vi "Initialize.vi"(7 "Configure RS232 Baud Rate":u32(ring)=115200 items=["9600"=9600, "19200"=19200, "38400"=38400, "57600"=57600, "115200"=115200], 8 "error in (no error)":errorcluster, 9 "Clear Error(True)":bool=TRUE, 10 "ID Query (True)":bool=TRUE, 11 "VISA resource name":refnum<visa-resource-name>) -> (0 "error out":errorcluster, 1 "ID Return Count":u32, 2 "ID Return String":string, 3 "VISA resource name out":refnum<visa-resource-name>)   [LabVIEW 2012, in "GDM-9052.lvlib"]
doc: "Establishes communication with the instrument and optionally performs an instrument identification query and/or an instrument reset. It also places the instrument in a default state needed for other instrument driver operations. Therefore, call this VI before calling other instrument driver VIs for this instrument. Generally, you need to call the Initialize VI only once at the beginning of an application."
uses:
  GDM-9052.lvlib
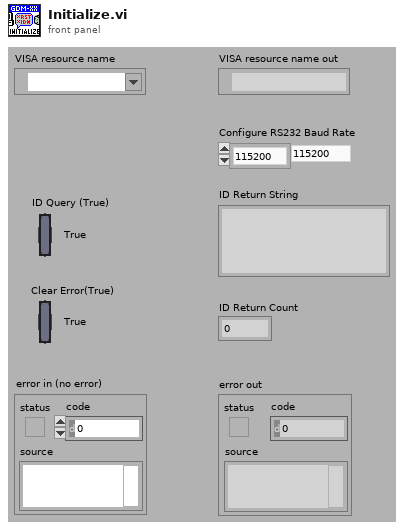
[diagram p1: front panel]
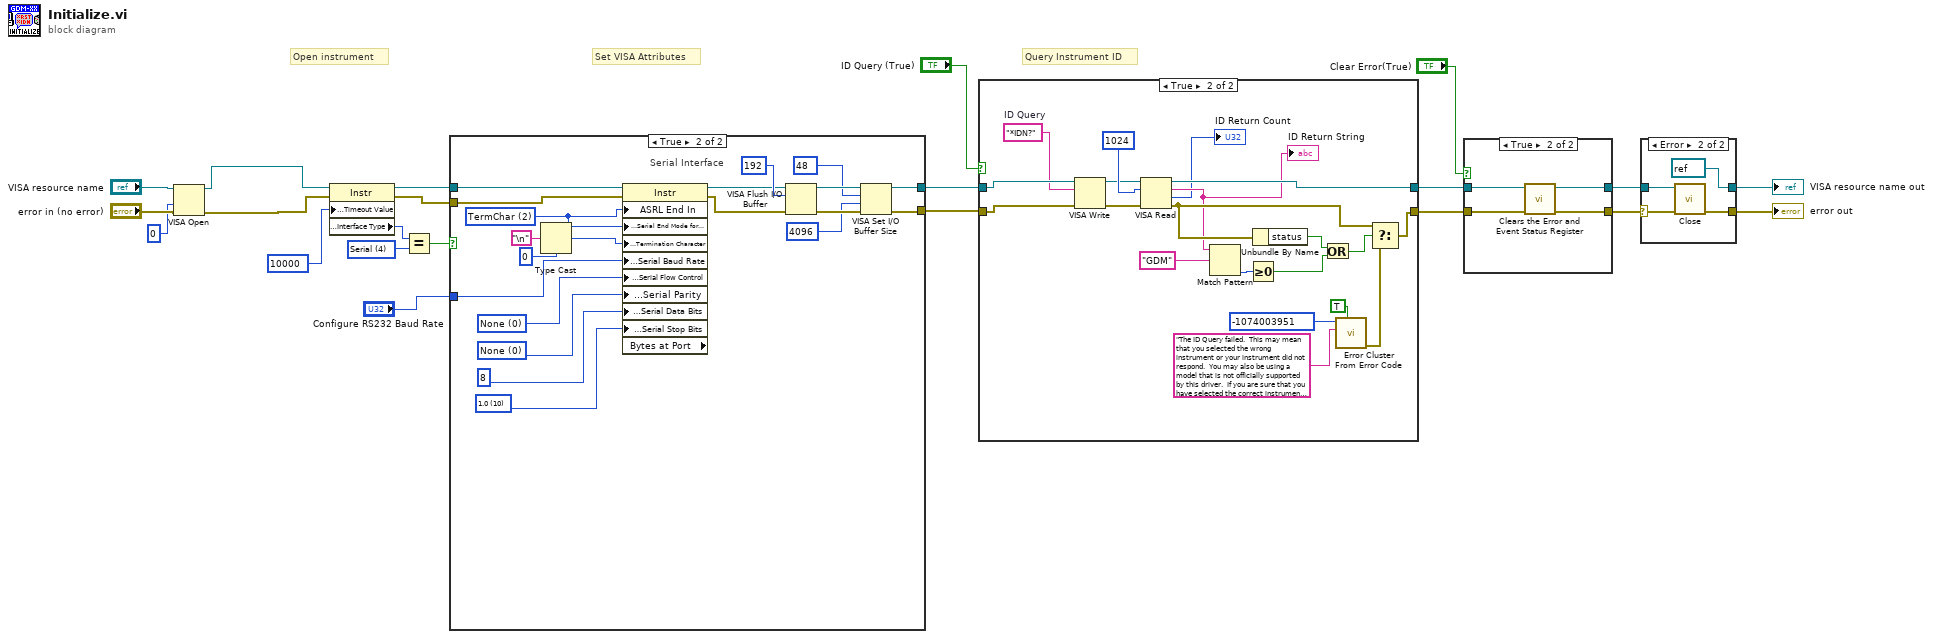
[diagram p0: block diagram]
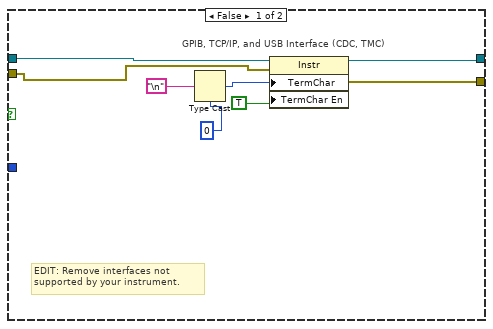
[diagram p4: hidden frame]
diagram:
  w14 = u16 4 items=["GPIB"=1, "VXI"=2, "GPIB-VXI"=3, "Serial"=4, "PXI"=5, "TCPIP"=6, "USB"=7] ("Interface Information:Interface Type")
  # "Set VISA Attributes"
  # "Query Instrument ID"
  # "Open instrument"
  n1 = VISA Open(access mode=u32 0, error in (no error)="error in (no error)", VISA resource name="VISA resource name") -> (VISA resource name=w5:refnum<visa-resource-name>, error out=w4:errorcluster)  [unwired: 2 in]
  n2 = property class="Instr"(reference=w5, error in=w4, "General Settings:Timeout Value"=u32 10000) -> (reference out=w17:refnum<visa-resource-name>, error out=w16:errorcluster, "Interface Information:Interface Type"=w11:u16)
  n3 = Equal?(x=w11, y=w14) -> (x = y?=w15:bool)
  n4 = case shown="True" w15 {
    tunnel: [w26 w32] -> w10
    tunnel: [w25 w31] -> w9
    tunnel: w17 -> [w24 w49]
    tunnel: w16 -> [w23 w50]
    tunnel: "Configure RS232 Baud Rate" -> [_ w36]
    frame False {
      # "GPIB, TCP/IP, and USB Interface (CDC, TMC)"
      # "EDIT: Remove interfaces not\nsupported by your instrument."
      n5 = Type Cast(type=u8 0, x="\n" ("Line Feed Constant")) -> (*(type *) &x=w30:u8)
      n6 = property class="Instr"(reference=w24, error in=w23, "TermChar"=w30, "TermChar En"=TRUE ("Message Based Settings:Termination Character Enable")) -> (reference out=w26:refnum<visa-resource-name>, error out=w25:errorcluster)
    }
    frame True {
      w39 = u16 10 items=["1.0"=10, "1.5"=15, "2.0"=20] ("Serial Settings:Stop Bits")
      w37 = u16 0 items=["None", "Odd", "Even", "Mark", "Space"] ("Serial Settings:Parity")
      w38 = u16 0 items=["None", "XON/XOFF", "RTS/CTS", "XON/XOFF & RTS/CTS", "DTR/DSR", "XON/XOFF & DTR/DSR"] ("Serial Settings:Flow Control")
      w35 = u16 2 items=["None", "LastBit", "TermChar"] ("Serial Settings:Serial End Mode for Reads")
      # "Serial Interface"
      n7 = Type Cast(type=u8 0, x="\n") -> (*(type *) &x=w41:u8)
      n8 = property class="Instr" props=["ASRL End In", "Serial Settings:Serial End Mode for Writes", "Message Based Settings:Termination Character", "Serial Settings:Serial Baud Rate", "Serial Settings:Serial Flow Control", "Serial Settings:Serial Parity", "Serial Settings:Serial Data Bits", "Serial Settings:Serial Stop Bits", "Bytes at Port"](reference=w49, error in=w50, "ASRL End In"=w35, "Serial Settings:Serial End Mode for Writes"=w35, "Message Based Settings:Termination Character"=w41, "Serial Settings:Serial Baud Rate"=w36, "Serial Settings:Serial Flow Control"=w38, "Serial Settings:Serial Parity"=w37, "Serial Settings:Serial Data Bits"=u16 8 ("Serial Settings:Data Bits"), "Serial Settings:Serial Stop Bits"=w39) -> (reference out=w34:refnum<visa-resource-name>, error out=w33:errorcluster)  [unwired: 1 out]
      n9 = VISA Flush I/O Buffer(VISA resource name=w34, mask (16)=u16 192, error in (no error)=w33) -> (VISA resource name out=w48:refnum<visa-resource-name>, error out=w47:errorcluster)
      n10 = VISA Set I/O Buffer Size(VISA resource name=w48, mask (16)=u16 48, size (4096)=u32 4096 ("size (0)"), error in (no error)=w47) -> (VISA resource name out=w32:refnum<visa-resource-name>, error out=w31:errorcluster)
    }
  }
  n11 = case shown="True" "ID Query (True)" {
    tunnel: [w51 w72] -> w21
    tunnel: [w52 w58] -> w22
    tunnel: w10 -> [w52 w61]
    tunnel: w9 -> [w51 w62]
    frame False {
    }
    frame True {
      w55 = "*IDN?"  # ID Query
      n12 = VISA Write(VISA resource name=w61, write buffer=w55, error in (no error)=w62) -> (VISA resource name out=w59:refnum<visa-resource-name>, error out=w57:errorcluster)  [unwired: 1 out]
      n13 = VISA Read(VISA resource name=w59, byte count=u32 1024, error in (no error)=w57) -> (VISA resource name out=w58:refnum<visa-resource-name>, read buffer=w54:string, return count=→"ID Return Count":u32, error out=w56:errorcluster)
      "ID Return String" <- w54
      n14 = Match Pattern(string=w54, regular expression="GDM") -> (offset past match=w66:i32)  [unwired: 1 in, 3 out]
      n15 = Greater Or Equal To 0?(x=w66) -> (x >= 0?=w64:bool)
      n16 = Unbundle By Name(w56) -> ("status"=w65:bool)
      n17 = Or(x=w65, y=w64) -> (x .or. y?=w63:bool)
      n18 = call <vilib>:"Error Cluster From Error Code.vi"("show call chain? (False)"=TRUE, "error message (\"\")"="The ID Query failed.  This may mean that you selected the wrong instrument or your instrument did not respond.  You may also be using a model that is not officially supported by this driver.  If you are sure that you have selected the correct instrument and it is responding, try disabling the ID Query." ("Source (VI Name)"), "error code (0)"=-1074003951 ("Code")) -> ("error out"=w70:errorcluster)  [unwired: 6 in]
      n19 = Select(t=w56, s=w63, f=w70) -> (s? t:f=w72:errorcluster)
    }
  }
  n20 = case shown="True" "Clear Error(True)" {
    tunnel: w21 -> [w73 w78]
    tunnel: [w73 w75] -> w1
    tunnel: w22 -> [w74 w77]
    tunnel: [w74 w76] -> w2
    frame False {
    }
    frame True {
      n21 = call "Clears the Error and Event Status Register.vi"("error in (no error)"=w78, "VISA resource name"=w77) -> ("error out"=w75:errorcluster, "VISA resource name out"=w76:refnum<visa-resource-name>)  [unwired: 8 in]
    }
  }
  n22 = case shown="Error" w1 {
    selector: w1 -> [w79 w82]
    tunnel: w2 -> [w80 w83]
    tunnel: [w80 refnum<visa-resource-name> refnum ("VISA resource name out")] -> w13
    tunnel: [w79 w84] -> w12
    frame No Error {
    }
    frame Error {
      n23 = call "Close.vi"("error in (no error)"=w82, "VISA resource name"=w83) -> ("error out"=w84:errorcluster)  [unwired: 9 in]
    }
  }
  "VISA resource name out" <- w13
  "error out" <- w12
